vi "Send Message.vi"(5 "return data? (F)":bool, 7 "action":T1, 8 "error in (no error)":errorcluster, 11 "send data":variant) -> (0 "error out":errorcluster, 3 "Variant":variant)   [LabVIEW 2018, in "GLog.lvlib" / "Registry.lvlib"]
uses:
  Registry.lvlib
  Registry Actions.ctl
  Registry Message.ctl
panel:
  # "Connector Pane"
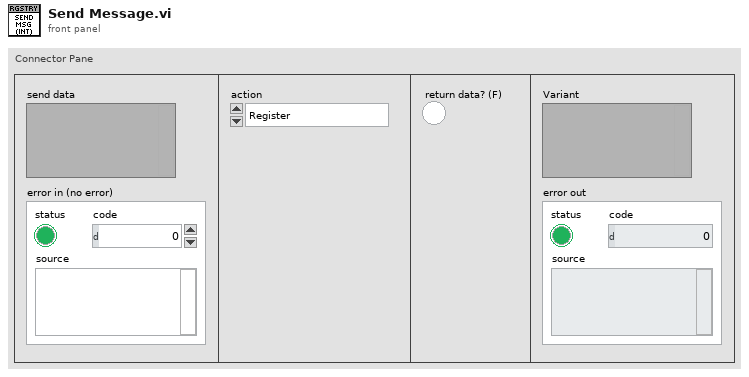
[diagram p1: front panel]
types:
  T1 = typedef "GLog.lvlib/Registry.lvlib/Registry Actions.ctl" = enum16{"Register", "Log", "Enable", "Enable All", "Disable", "Disable All", "Get Enable State", "Get Minimum Log Level", "Set Minimum Log Level", "Set All Minimum Log Level", "Get Logger Info", "Get All Logger Info", "List", "Unregister", "Unregister All", "Shutdown"}
  T2 = typedef "GLog.lvlib/Registry.lvlib/Registry Message.ctl" = cluster{"action":T1, "data":variant, "return notifier":refnum<notifier>}
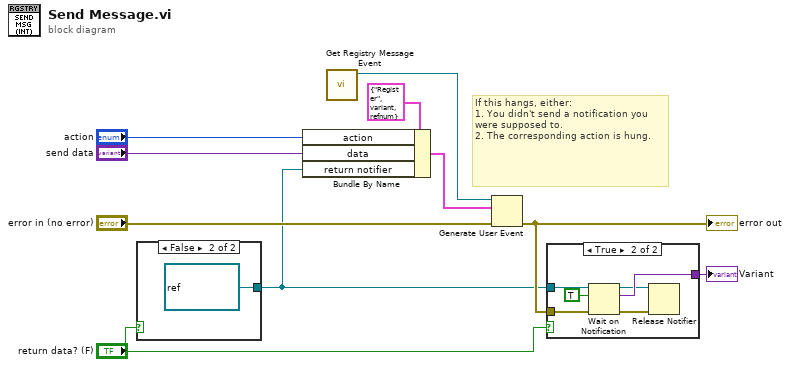
[diagram p0: block diagram]
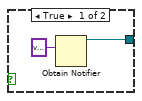
[diagram p2: hidden frame]
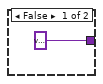
[diagram p3: hidden frame]
diagram:
  # "If this hangs, either:\n1. You didn't send a notification you were supposed to.\n2. The corresponding action is hung."
  n1 = case shown="False" "return data? (F)" {
    tunnel: [w12 refnum<notifier> refnum ("notifier out")] -> w6
    frame True {
      n2 = Obtain Notifier(notification data type=variant ("element data type")) -> (notifier out=w12:refnum<notifier>)  [unwired: 3 in, 2 out]
    }
    frame False {
    }
  }
  n3 = Bundle By Name(cluster=T2 {"action"=enum."Register", "data"=variant, "return notifier"=refnum} ("registry message"), "action"="action", "data"="send data", "return notifier"=w6) -> (w4:T2)
  n4 = call "Get Registry Message Event.vi"() -> ("registry message event"=w7:refnum<user-event>)  [unwired: 11 in]
  n5 = Generate User Event(user event=w7, event data cluster=w4, error in="error in (no error)") -> (error out=w8:errorcluster)  [unwired: 1 in, 1 out]
  "error out" <- w8
  n6 = case shown="True" "return data? (F)" {
    tunnel: w6 -> [_ w20]
    tunnel: [variant w19] -> w2
    tunnel: w8 -> [_ w16]
    frame False {
    }
    frame True {
      n7 = Wait on Notification(notifier=w20, ignore previous (F)=TRUE, error in (no error)=w16) -> (notifier out=w18:refnum<notifier>, notification=w19:variant, error out=w15:errorcluster)  [unwired: 1 in, 1 out]
      n8 = Release Notifier(notifier=w18, error in (no error)=w15) -> ()  [unwired: 1 in, 3 out]
    }
  }
  "Variant" <- w2
